vi "Set Queue Attributes.vi"(8 "error in (no error)":errorcluster, 10 "Attributes":T1[](array[typedef]), 11 "SQS in":refnum<class "Queue.lvclass">) -> (0 "error out":errorcluster, 3 "SQS out":refnum<class "Queue.lvclass">)   [LabVIEW 2015, in "NI_AWS_SQS.lvlib" / "Queue.lvclass"]
doc: "Sets the value of one or more queue attributes. When you change a queue's attributes, the change can take up to 60 seconds for most of the attributes to propagate throughout the Amazon SQS system. Changes made to the MessageRetentionPeriod attribute can take up to 15 minutes."
uses:
  Queue.lvclass
  Queue Attribute Value Pair.ctl
  Queue Attribute.ctl
  Core/HTTP Request/Name Value Pair.ctl
  Core/HTTP Request/Request Options.ctl
  Core/HTTP Request/Region handling.ctl
  Core/HTTP Request/URL formatting.ctl
  Queue.lvclass/Queue.ctl
  Read Account Number.vi
  Read Name.vi
  Core/HTTP Request/HTTP Request.lvclass
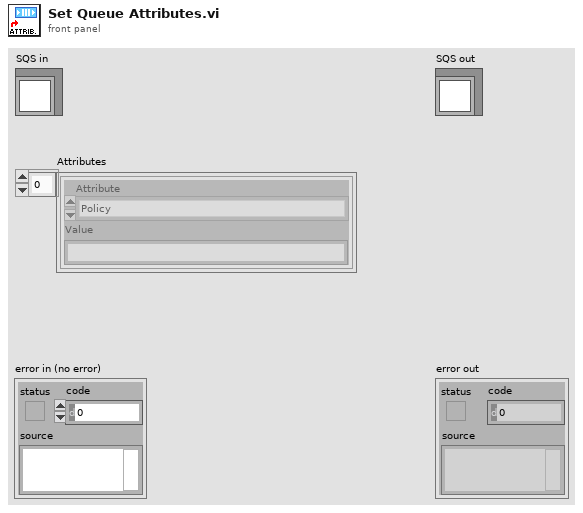
[diagram p1: front panel]
types:
  T1 = typedef "NI_AWS_SQS.lvlib/Queue.lvclass/Queue Attribute Value Pair.ctl" = cluster{"Attribute":T2, "Value":string}
  T2 = typedef "NI_AWS_SQS.lvlib/Queue.lvclass/Queue Attribute.ctl" = enum16{"ApproximateNumberOfMessages", "ApproximateNumberOfMessagesDelayed", "ApproximateNumberOfMessagesNotVisible", "CreatedTimestamp", "DelaySeconds", "LastModifiedTimestamp", "MaximumMessageSize", "MessageRetentionPeriod", "Policy", "QueueArn", "ReceiveMessageWaitTimeSeconds", "RedrivePolicy", "VisibilityTimeout"}
  T3 = typedef "NI_AWS_Core.lvlib/HTTP Request.lvclass/Request Options.ctl" = cluster{"request headers":T4[], "request parameters":T4[], "request body":string, "region handling":T5, "URL formatting":T6}
  T4 = typedef "NI_AWS_Core.lvlib/HTTP Request.lvclass/Name Value Pair.ctl" = cluster{"name":string, "value":string}
  T5 = typedef "NI_AWS_Core.lvlib/HTTP Request.lvclass/Region handling.ctl" = enum16{"use region everywhere", "use region (authentication only)", "use region (URL only)", "ignore region everwhere"}
  T6 = typedef "NI_AWS_Core.lvlib/HTTP Request.lvclass/URL formatting.ctl" = enum16{"region-", "region."}
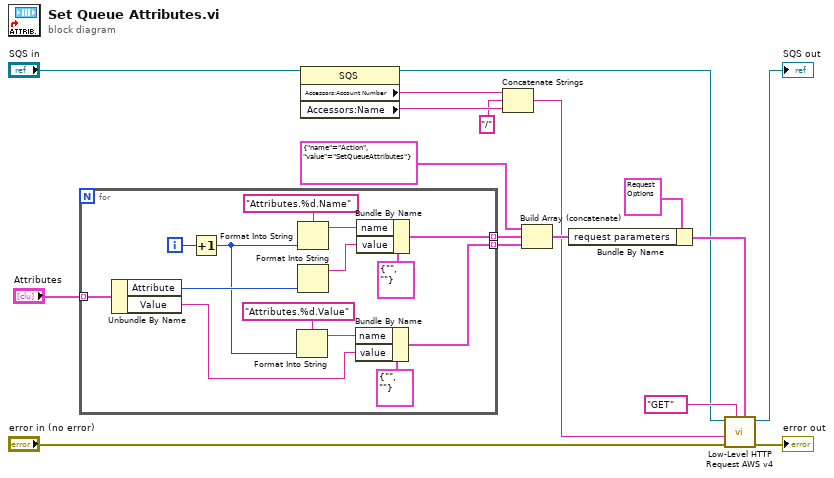
[diagram p0: block diagram]
diagram:
  n1 = for {
    tunnel: "Attributes" -> [w26] mode=indexing
    tunnel: [w27] -> w11 mode=indexing
    tunnel: [w20] -> w5 mode=indexing
    i -> [w31]
    n2 = Unbundle By Name(w26) -> ("Attribute"=w24:T2, "Value"=w18:string)
    n3 = Increment(x=w31) -> (x+1=w19:i32)
    n4 = Format Into String(format string="Attributes.%d.Value", w19) -> (resulting string=w23:string)  [unwired: 2 in, 1 out]
    n5 = Format Into String(format string="Attributes.%d.Name", w19) -> (resulting string=w28:string)  [unwired: 2 in, 1 out]
    n6 = Format Into String(w24) -> (resulting string=w25:string)  [unwired: 3 in, 1 out]
    n7 = Bundle By Name(cluster=T4 {"name"="", "value"=""} ("element"), "name"=w23, "value"=w18) -> (w20:T4)
    n8 = Bundle By Name(cluster=T4 {"name"="", "value"=""} ("element"), "name"=w28, "value"=w25) -> (w27:T4)
  }
  n9 = property class="SQS"(reference="SQS in") -> (reference out=w1:refnum<class "Queue.lvclass">, "Accessors:Account Number"=w10:string, "Accessors:Name"=w9:string)  [unwired: 1 in, 1 out]
  n10 = Concatenate Strings(w10, "/", w9) -> (w7:string)
  n11 = Build Array (concatenate)(T4 {"name"="Action", "value"="SetQueueAttributes"} ("Cluster"), w11, w5) -> (w12:T4[])
  n12 = Bundle By Name(cluster=T3 {"request headers"=[], "request parameters"=[{"name"="Action", "value"="ListQueues"}], "request body"="", "region handling"=enum."use region everywhere", "URL formatting"=enum."region."} ("Request Options"), "request parameters"=w12) -> (w3:T3)
  n13 = call "Low-Level HTTP Request AWS v4.vi"("Request Options"=w3, "HTTP-Verb"="GET", "error in (no error)"="error in (no error)", "URL Suffix"=w7, "AWS Core in"=w1) -> ("error out"=→"error out":errorcluster, "AWS Core out"=→"SQS out":refnum<class "Queue.lvclass">)  [unwired: 3 in, 2 out]
